vi "Notifier_Manager.vi"(0 "Notifier Data":variant, 2 "Notifier Name":T1=enum."Test", 11 "Error In":errorcluster, 13 "Notifier Options":T2) -> (4 "Notifier Data":variant, 15 "Error Out":errorcluster)   [LabVIEW 2026, in "Core.lvlib"]
doc: "Manages notifier references and associated data."
uses:
  Core.lvlib
  TypeDefs/Enum_Notifier_Options.ctl
  TypeDefs/Enum_Notifier_Name.ctl
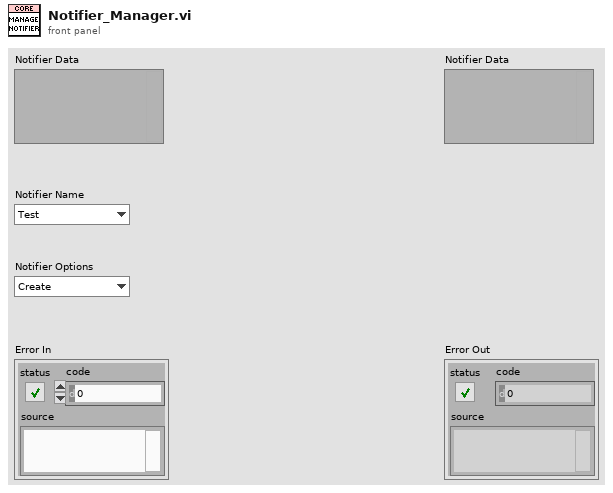
[diagram p1: front panel]
types:
  T1 = typedef "Core.lvlib/Enum_Notifier_Name.ctl" = enum16{"Device Type", "Test", "Instrument Spec", "Measurement Spec", "Status"}
  T2 = typedef "Core.lvlib/Enum_Notifier_Options.ctl" = enum16{"Create", "Send", "Status", "Release"}
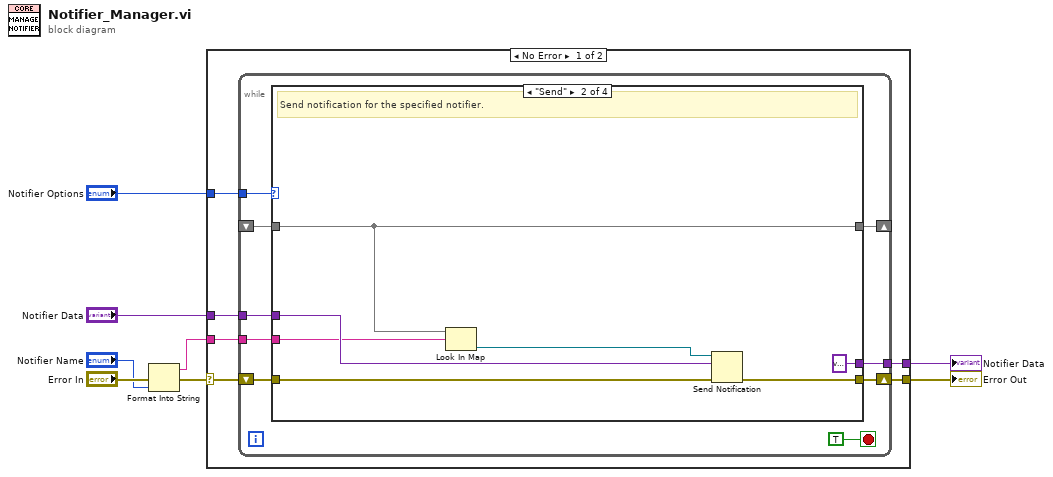
[diagram p0: block diagram]
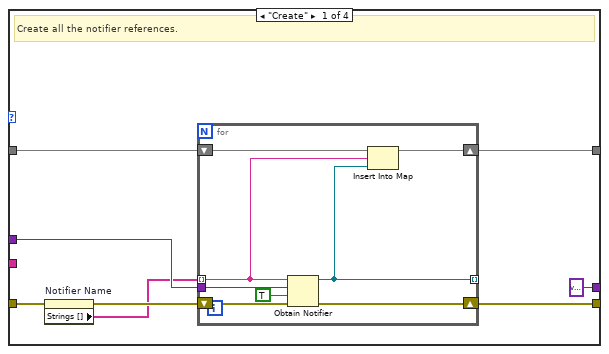
[diagram p2: hidden frame]
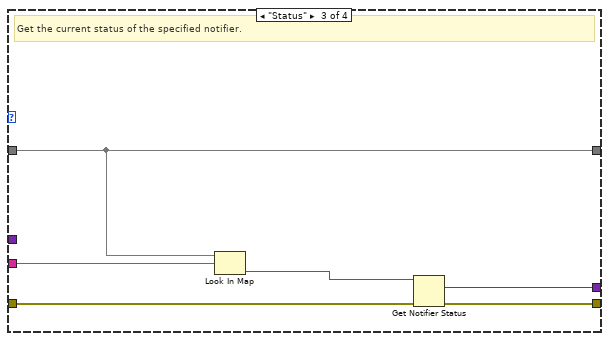
[diagram p3: hidden frame]
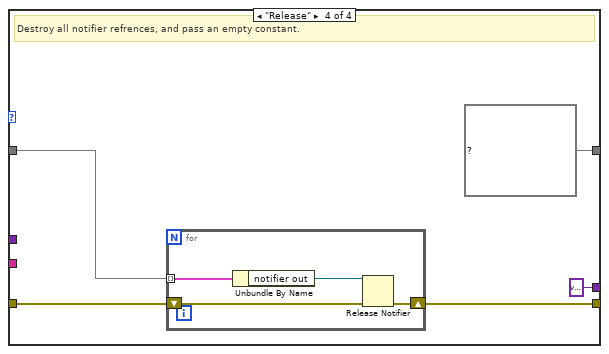
[diagram p4: hidden frame]
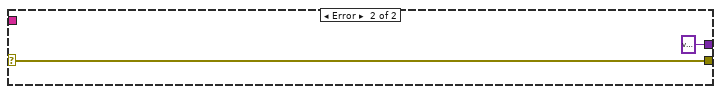
[diagram p5: hidden frame]
diagram:
  n1 = Format Into String(error in="Error In", "Notifier Name") -> (resulting string=w2:string, error out=w4:errorcluster)  [unwired: 2 in]
  n2 = case shown="No Error" w4 {
    selector: w4 -> [w14 w63]
    tunnel: "Notifier Options" -> [w13 _]
    tunnel: [w12 w63] -> w6
    tunnel: "Notifier Data" -> [w11 _]
    tunnel: w2 -> [w10 _]
    tunnel: [w9 variant ("Variant")] -> w1
    frame No Error {
      n3 = while {
        tunnel: w13 -> [w22]
        shift-right: [w20] -> w12
        shift-left: w14 -> [w21]
        shift-right: [w15] -> _
        shift-left: _ -> [w16]
        tunnel: w11 -> [w19]
        tunnel: w10 -> [w18]
        tunnel: [w17] -> w9
        stop <- TRUE stop-if-true
        n4 = case shown="\"Send\"" w22 {
          tunnel: w21 -> [w31 w44 w52 w57]
          tunnel: [w30 w46 w51 w56] -> w20
          tunnel: w19 -> [w29 w45 _ _]
          tunnel: w18 -> [_ w42 w50 _]
          tunnel: [variant ("Variant") variant ("Variant") w47 variant ("Variant")] -> w17
          tunnel: w16 -> [w27 w40 w48 w53]
          tunnel: [w26 w40 w48 map{string, refnum<notifier>} {} ("map")] -> w15
          frame "Create" {
            # "Create all the notifier references."
            n5 = property on="Notifier Name" class="Enum (strict)"(error in=w31) -> (error out=w25:errorcluster, "Strings []"=w24:string[])  [unwired: 1 in, 1 out]
            n6 = for {
              shift-right: [w38] -> w30
              shift-left: w25 -> [w39]
              tunnel: [w33] -> _ mode=indexing
              tunnel: w29 -> [w35]
              tunnel: w24 -> [w32] mode=indexing
              shift-right: [w34] -> w26
              shift-left: w27 -> [w36]
              n7 = Obtain Notifier(name (unnamed)=w32, notification data type=w35, create if not found? (T)=TRUE, error in (no error)=w39) -> (notifier out=w33:refnum<notifier>, error out=w38:errorcluster)  [unwired: 1 out]
              n8 = Insert Into Map(map in=w36, key=w32, value=w33) -> (map out=w34:map{string, refnum<notifier>})  [unwired: 2 out]
            }
          }
          frame "Send" {
            # "Send notification for the specified notifier."
            n9 = Look In Map(map=w40, key=w42) -> (value=w41:refnum<notifier>)  [unwired: 1 in, 1 out]
            n10 = Send Notification(notification=w45, notifier=w41, error in (no error)=w44) -> (error out=w46:errorcluster)  [unwired: 1 out]
          }
          frame "Status" {
            # "Get the current status of the specified notifier."
            n11 = Look In Map(map=w48, key=w50) -> (value=w49:refnum<notifier>)  [unwired: 1 in, 1 out]
            n12 = Get Notifier Status(notifier=w49, error in (no error)=w52) -> (current notification=w47:variant, error out=w51:errorcluster)  [unwired: 3 out]
          }
          frame "Release" {
            # "Destroy all notifier refrences, and pass an empty constant."
            n13 = for {
              shift-right: [w60] -> w56
              shift-left: w57 -> [w61]
              tunnel: w53 -> [w59] mode=indexing
              n14 = Unbundle By Name(w59) -> ("notifier out"=w58:refnum<notifier>)
              n15 = Release Notifier(notifier=w58, error in (no error)=w61) -> (error out=w60:errorcluster)  [unwired: 1 in, 2 out]
            }
          }
        }
      }
    }
    frame Error {
    }
  }
  "Error Out" <- w6
  "Notifier Data" <- w1
